vi "BNO055 READ.vi"(8 "error IN":errorcluster, 11 "I2C Ref Out":T1) -> (2 "Yaw":dbl, 3 "Degrees":cluster{"Yaw":dbl, "Roll":dbl, "Pitch":dbl})   [LabVIEW 2019]
uses:
  <vilib>/myRIO/Instrument Drivers/Onboard IO/I2C/typedefs/I2C Reference.ctl
  <vilib>/myRIO/Common/Instrument Driver Framework/Utilities/typedefs/myRIO Generic Hardware Reference.ctl
  <vilib>/myRIO/Common/Instrument Driver Framework/Utilities/typedefs/Hardware Version Enum.ctl
  <vilib>/myRIO/Common/Instrument Driver Framework/Utilities/typedefs/myRIO v1.0 Reference.ctl
  <vilib>/myRIO/Common/Instrument Driver Framework/Utilities/typedefs/Generic FPGA Reference.ctl
  <vilib>/myRIO/Common/Instrument Driver Framework/myRIO v1.0/I2C/typedefs/I2C Channels Enum.ctl
  <vilib>/myRIO/Instrument Drivers/Onboard IO/I2C/typedefs/I2C Configuration.ctl
  <vilib>/myRIO/Instrument Drivers/Onboard IO/I2C/typedefs/I2C Transfer Rate.ctl
  <vilib>/Utility/error.llb/Error Cluster From Error Code.vi
  <vilib>/myRIO/Common/Instrument Driver Framework/myRIO v1.0/I2C/vis/myRIO v1.0 Write I2C.vi
  <vilib>/myRIO/Common/Instrument Driver Framework/myRIO v1.0/I2C/vis/myRIO v1.0 Read I2C.vi
  <vilib>/myRIO/Instrument Drivers/Onboard IO/I2C/I2C.lvlib
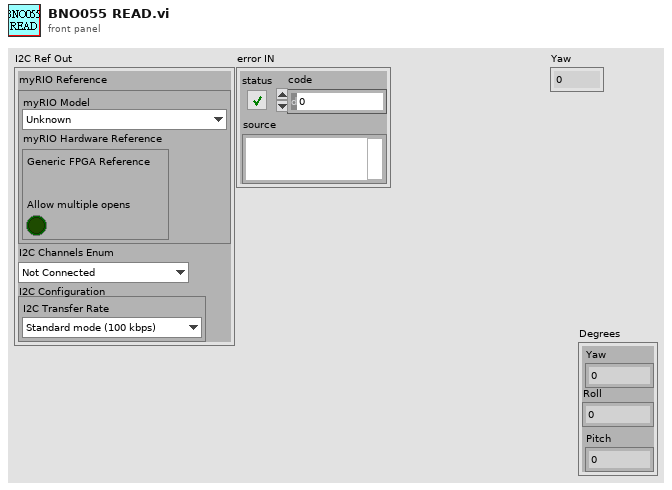
[diagram p1: front panel]
types:
  T1 = typedef "I2C.lvlib/I2C Reference.ctl" = cluster{"myRIO Reference":T2, "I2C Channels Enum":T6, "I2C Configuration":T7}
  T2 = typedef "myRIO Generic Hardware Reference.ctl" = cluster{"myRIO Model":T3, "myRIO Hardware Reference":T4}
  T3 = typedef "Hardware Version Enum.ctl" = enum16{"Unknown", "myRIO-1900", "myRIO-1950", "roboRIO", "NI ELVIS RIO CM", "ELVIS III"}
  T4 = typedef "myRIO v1.0 Reference.ctl" = cluster{"Generic FPGA Reference":T5, "Allow multiple opens":bool}
  T5 = typedef "Generic FPGA Reference.ctl" = refnum<k20>
  T6 = typedef "I2C Channels Enum.ctl" = enum16{"Not Connected", "A/I2C", "B/I2C", "I2C/I2C"}
  T7 = typedef "I2C.lvlib/I2C Configuration.ctl" = cluster{"I2C Transfer Rate":T8}
  T8 = typedef "I2C.lvlib/I2C Transfer Rate.ctl" = enum16{"Standard mode (100 kbps)", "Fast mode (400 kbps)"}
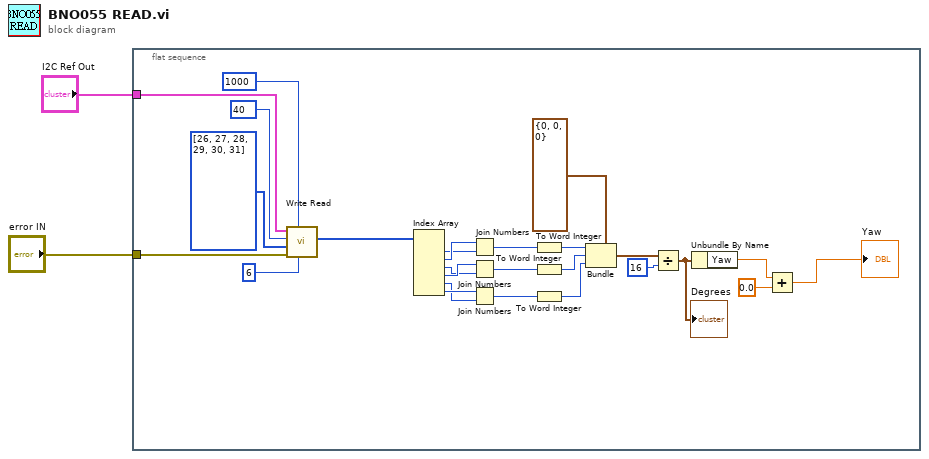
[diagram p0: block diagram]
diagram:
  n1 = flat-sequence {
    tunnel: "error IN" -> [w28]
    tunnel: "I2C Ref Out" -> [w27]
    frame #0 {
      n2 = call <vilib>:"Write Read.vi"("Byte Count"=u32 6, "Timeout ms (1000)"=1000, "error in (no error)"=w28, "Bytes to Write"=i32[] [26, 27, 28, 29, 30, 31], "Slave Address (7-bit)"=40, "I2C Ref In"=w27) -> ("Bytes Read"=w22:u8[])  [unwired: 2 in, 2 out]
      n3 = Index Array(array=w22) -> (element #1=w20:u8, element #2=w21:u8, element #3=w18:u8, element #4=w19:u8, element #5=w16:u8, element #6=w17:u8)  [unwired: 6 in]
      n4 = Join Numbers(hi=w21, lo=w20) -> ((hi.lo)=w15:u16)
      n5 = Join Numbers(hi=w19, lo=w18) -> ((hi.lo)=w14:u16)
      n6 = Join Numbers(hi=w17, lo=w16) -> ((hi.lo)=w13:u16)
      n7 = To Word Integer(number=w15) -> (16bit integer=w12:i16)
      n8 = To Word Integer(number=w14) -> (16bit integer=w11:i16)
      n9 = To Word Integer(number=w13) -> (16bit integer=w10:i16)
      n10 = Bundle(cluster=cluster{"Yaw":i16, "Roll":i16, "Pitch":i16} {"Yaw"=0, "Roll"=0, "Pitch"=0}, "Yaw"=w12, "Roll"=w11, "Pitch"=w10) -> (w8:cluster{"Yaw":i16, "Roll":i16, "Pitch":i16})
      n11 = Divide(x=w8, y=u32 16 ("Byte Count")) -> (x/y=w6:cluster{"Yaw":dbl, "Roll":dbl, "Pitch":dbl})
      "Degrees" <- w6
      n12 = Unbundle By Name(w6) -> ("Yaw"=w5:dbl)
      n13 = Add(x=w5, y=0.0) -> (x+y=→"Yaw":dbl)
    }
  }
